vi "SA get Trace Data.vi"(8 "error in (no error)":errorcluster caption="에러 입력(에러 없음)", 11 "Instrument Manager 입력":refnum<class "Instrument Manager.lvclass">) -> (0 "error out":errorcluster caption="에러 출력", 2 "Trace Values":T1 {"Frequency" format="%#_6p"}, 3 "Instrument Manager 출력":refnum<class "Instrument Manager.lvclass">)   [LabVIEW 2023, in "Instrument Manager.lvclass"]
uses:
  Instrument Manager.lvclass
  Module/Spectrum Analyzer/TYPE DEFINITION/TYPE Trace Value Array.ctl
  Instrument Manager.lvclass/Instrument Manager.ctl
  Module/Spectrum Analyzer/Interface_Spectrum/Interface_Spectrum.lvclass
  Module/Spectrum Analyzer/Spectrum Analyzer.lvlib
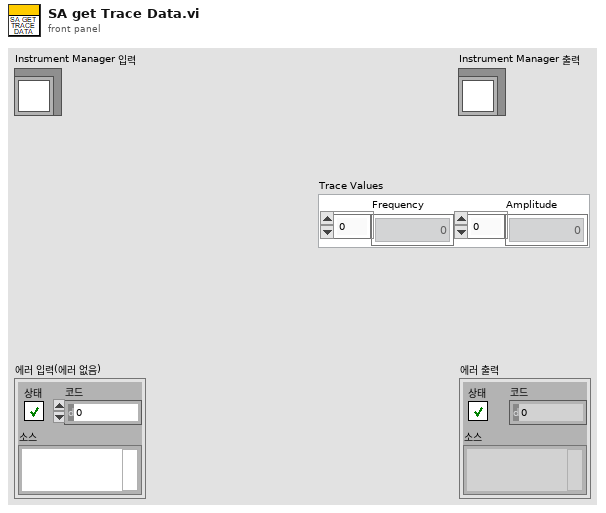
[diagram p1: front panel]
types:
  T1 = typedef "Spectrum Analyzer.lvlib/TYPE Trace Value Array.ctl" = cluster{"Frequency":dbl[], "Amplitude":dbl[]}
  T2 = cluster{"Anritsu Call Box":refnum<class "Anritsu Call Box.lvclass">, "Spectrum Analyzer":refnum<class "Interface_Spectrum.lvclass">, "RF Switch Box":refnum<class "RF Filter Box.lvclass">, "Turn Table":refnum<class "Interface - Turn Table.lvclass">, "Mast":refnum<class "Interface - Mast.lvclass">, "3D Controller":refnum<class "Interface_3D Controller.lvclass">}
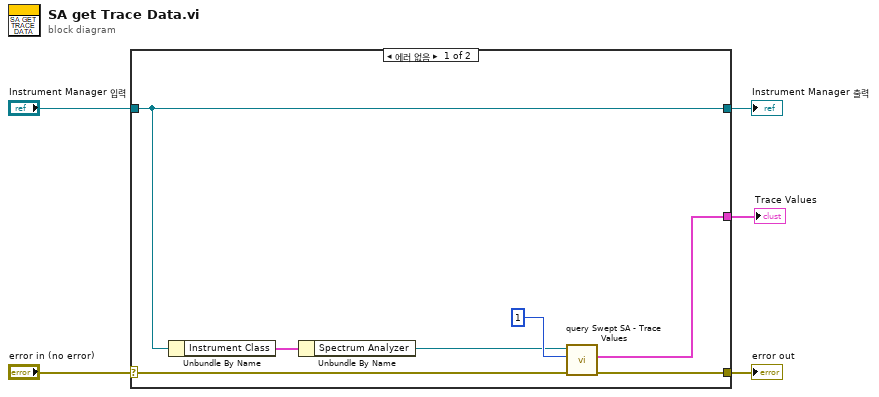
[diagram p0: block diagram]
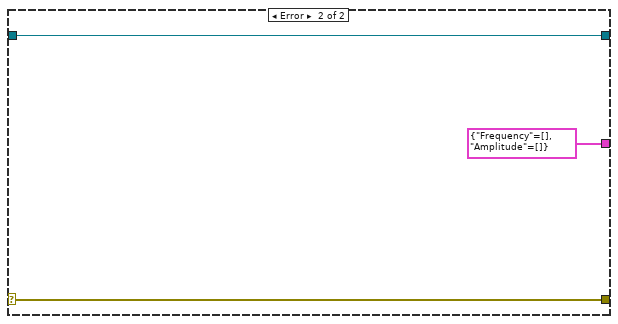
[diagram p2: hidden frame]
diagram:
  n1 = case shown="에러 없음" "error in (no error)" {
    selector: "error in (no error)" -> [w6 w15]
    tunnel: [w9 w15] -> w4
    tunnel: [w12 w14] -> w2
    tunnel: "Instrument Manager 입력" -> [w12 w14]
    tunnel: [w8 T1 {"Frequency"=[], "Amplitude"=[]} ("Trace Values")] -> w1
    frame No Error {
      n2 = Unbundle By Name(w12) -> ("Instrument Class"=w11:T2)
      n3 = Unbundle By Name(w11) -> ("Spectrum Analyzer"=w7:refnum<class "Interface_Spectrum.lvclass">)
      n4 = call-dynamic "query Swept SA - Trace Values.vi"("error in (no error)"=w6, "Trace Index"=u32 1, "Interface_Spectrum in"=w7) -> ("error out"=w9:errorcluster, "Trace Values"=w8:T1)  [unwired: 6 in, 1 out]
    }
    frame Error {
    }
  }
  "error out" <- w4
  "Instrument Manager 출력" <- w2
  "Trace Values" <- w1
